vi "Create Instance.vi"(8 "error in":errorcluster, 10 "parameters":refnum<k24>[](array[refnum]), 11 "Runtime Type":refnum<k24>) -> (0 "error out":errorcluster, 3 "Instance":refnum<k24>)   [LabVIEW 2026, in "ToastNotification.lvlib" / "Reflection DotNet.lvlib"]
doc: "Create a runtime object with Activator.CreateInstance(Type, Object[]). Borrow Runtime Type and constructor parameters. Skipped on incoming error. Caller owns Instance, including a valid result returned with an error. Does not close the borrowed arguments."
uses:
  Reflection DotNet.lvlib
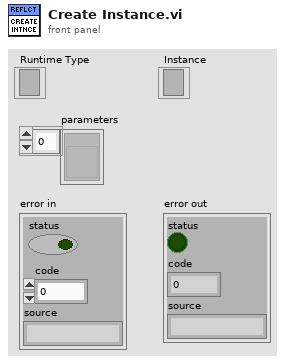
[diagram p1: front panel]
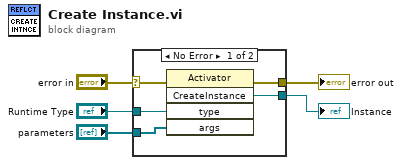
[diagram p0: block diagram]
diagram:
  n1 = case shown="No Error" "error in" {
    selector: "error in" -> [w6 w11]
    tunnel: "Runtime Type" -> [w7 _]
    tunnel: "parameters" -> [w8 _]
    tunnel: [w9 _] -> w4
    tunnel: [w10 w11] -> w5
    frame No Error {
      n2 = invoke class="Activator" method="CreateInstance"(error in=w6, "type"=w7, "args"=w8) -> (error out=w10:errorcluster, "CreateInstance"=w9:refnum<k24>)  [unwired: 2 in, 3 out]
    }
    frame Error {
    }
  }
  "Instance" <- w4
  "error out" <- w5
